vi "Document_AddContent.vi"(8 "error in (no error)":errorcluster, 10 "Content":refnum<k24>, 11 "ooWriter in":refnum<class "ooWriter.lvclass">) -> (0 "error out":errorcluster, 3 "ooWriter out":refnum<class "ooWriter.lvclass">)   [LabVIEW 2009, in "ooWriter.lvclass"]
uses:
  ooWriter.lvclass
  C:/Projets/LAVAG/OpenOfficeRGT/AODL/DLLs/AODL.dll
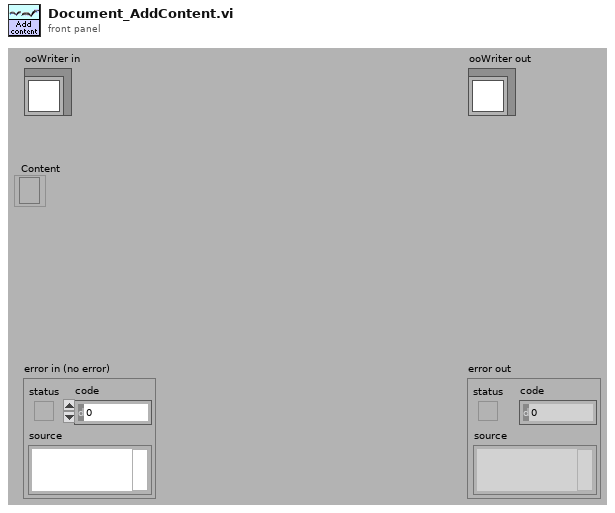
[diagram p1: front panel]
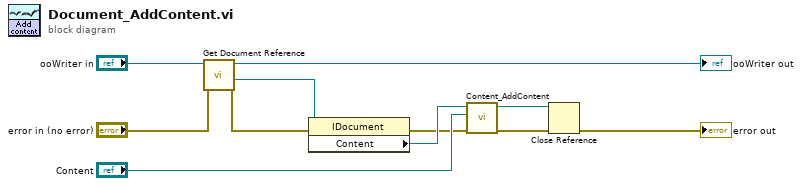
[diagram p0: block diagram]
diagram:
  n1 = call-dynamic "Get Document Reference.vi"("error in (no error)"="error in (no error)", "ooDocument in"="ooWriter in") -> ("error out"=w3:errorcluster, "Document"=w4:refnum<k24>, "ooDocument out"=→"ooWriter out":refnum<class "ooWriter.lvclass">)  [unwired: 7 in]
  n2 = property class="IDocument"(reference=w4, error in=w3) -> (error out=w5:errorcluster, "Content"=w6:refnum<k24>)  [unwired: 1 out]
  n3 = call "Content_AddContent.vi"("error in"=w5, "Content"="Content", "ContentCollection"=w6) -> ("error out"=w1:errorcluster, "ContentCollection dup"=w2:refnum<k24>)  [unwired: 7 in]
  n4 = Close Reference(reference=w2, error in (no error)=w1) -> (error out=→"error out":errorcluster)
